vi "Lidar_obstacle.vi"(8 "error in (no error)":errorcluster, 10 "Enum Zone":T1, 11 "Tableau lidar":dbl[][](array[numeric])=[[0.0, 1.0, 2.0, 3.0, 4.0, 5.0, 6.0, 7.0, 8.0, 9.0, 10.0, 11.0, 12.0, 13.0, 14.0, 15.0, 16.0, 17.0, 18.0, 19.0, 20.0, 21.0, 22.0, 23.0, 24.0, 25.0, 26.0, 27.0, 28.0, 29.0, 30.0, 31.0, 32.0, 33.0, 34.0, 35.0], [20.0, 15.0, 30.0, 31.0, 42.0, 50.0, 51.0, 60.0, 20.0, 15.0, 30.0, 31.0, 42.0, 50.0, 51.0, 60.0, 20.0, 15.0, 30.0, 31.0, 42.0, 50.0, 51.0, 60.0, 20.0, 15.0, 30.0, 31.0, 42.0, 50.0, 51.0, 60.0, 20.0, 15.0, 30.0, 31.0], [0.0, 0.0, 0.0, 0.0, 0.0, 0.0, 0.0, 0.0, 0.0, 0.0, 0.0, 0.0, 0.0, 0.0, 0.0, 0.0, 0.0, 0.0, 0.0, 0.0, 0.0, 0.0, 0.0, 0.0, 0.0, 0.0, 0.0, 0.0, 0.0, 0.0, 0.0, 0.0, 0.0, 0.0, 0.0, 0.0]]) -> (0 "error out":errorcluster, 1 "Zone 2":dbl[][](array[numeric]), 2 "Zone 3":dbl[][](array[numeric]), 3 "Espace libre":dbl[][](array[numeric]))   [LabVIEW 2018]
uses:
  enum_zone.ctl
panel:
  out "Espace libre sans angle visé":dbl[][](array[numeric])
  out "Index ZM":i32
  out "Ecart superieur Alpha":dbl[][](array[numeric])
  out "Zone 3 bis + limite ZM":dbl[][](array[numeric])
  out "initialized array ecart":dbl[][](array[numeric])
  out "Zone 3 Bis":dbl[][](array[numeric])
  out "Detec part 3":dbl[][](array[numeric])
  out "Nbr ° à enlever début 2":i32
  out "Nbr ° à enlever fin 2":i32
  out "Début detec 3":i32
  out "Detec part 4":dbl[][](array[numeric])
  out "Moitié de Alpha":dbl
  in  "Alpha":i32=90
  in  "L2":dbl=30.0
  in  "L3":dbl=60.0
  out "Zone de detection":dbl[][](array[numeric])
  out "Nbr ° à enlever fin":dbl
  out "Début detec 2":dbl
  out "Detec part 2":dbl[][](array[numeric])
  out "Nbr ° à enlever début":dbl
  out "Detec part 1":dbl[][](array[numeric])
  out "Moitié de ZM":dbl
  in  "Angle zone morte (°)":i32=180
  out "Angles / distance / statut":dbl[][](array[numeric])
  # "Face Avant"
  # "Debug"
  # "Zone morte retirée"
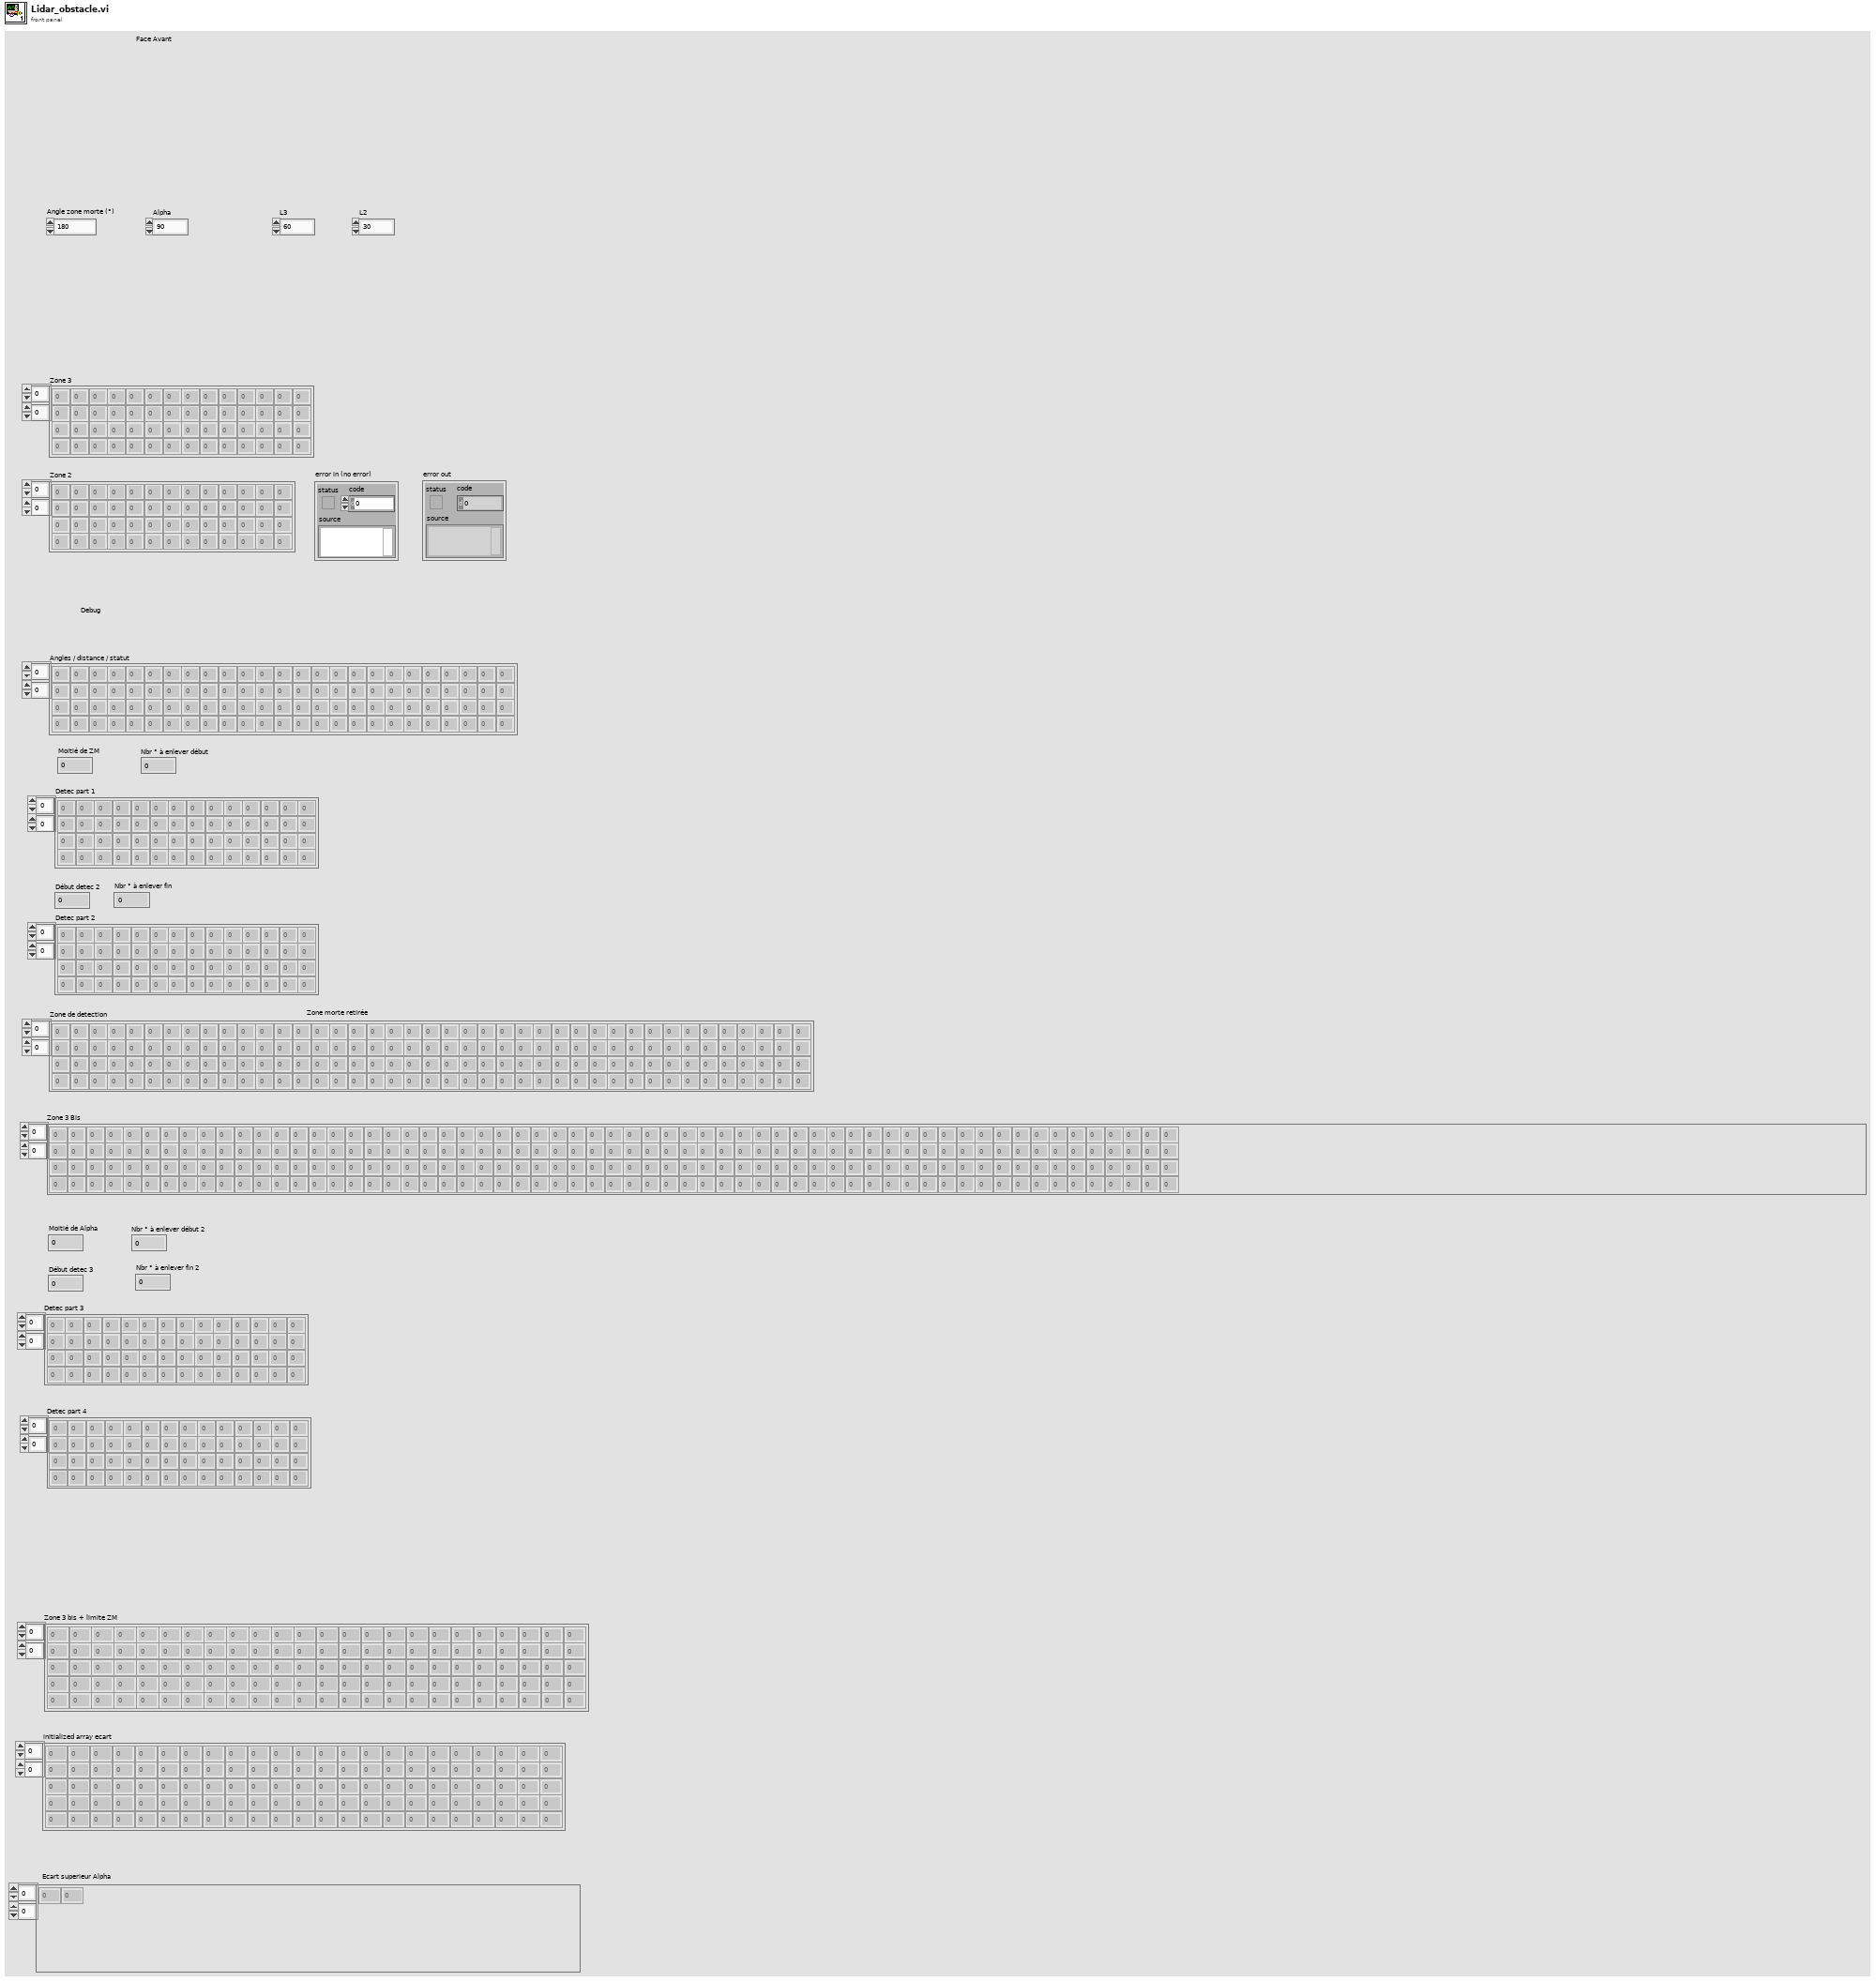
[diagram p1: front panel]
types:
  T1 = typedef "enum_zone.ctl" = enum16{"Zone_2", "Zone_3", "Espace_libre", "Aucune"}
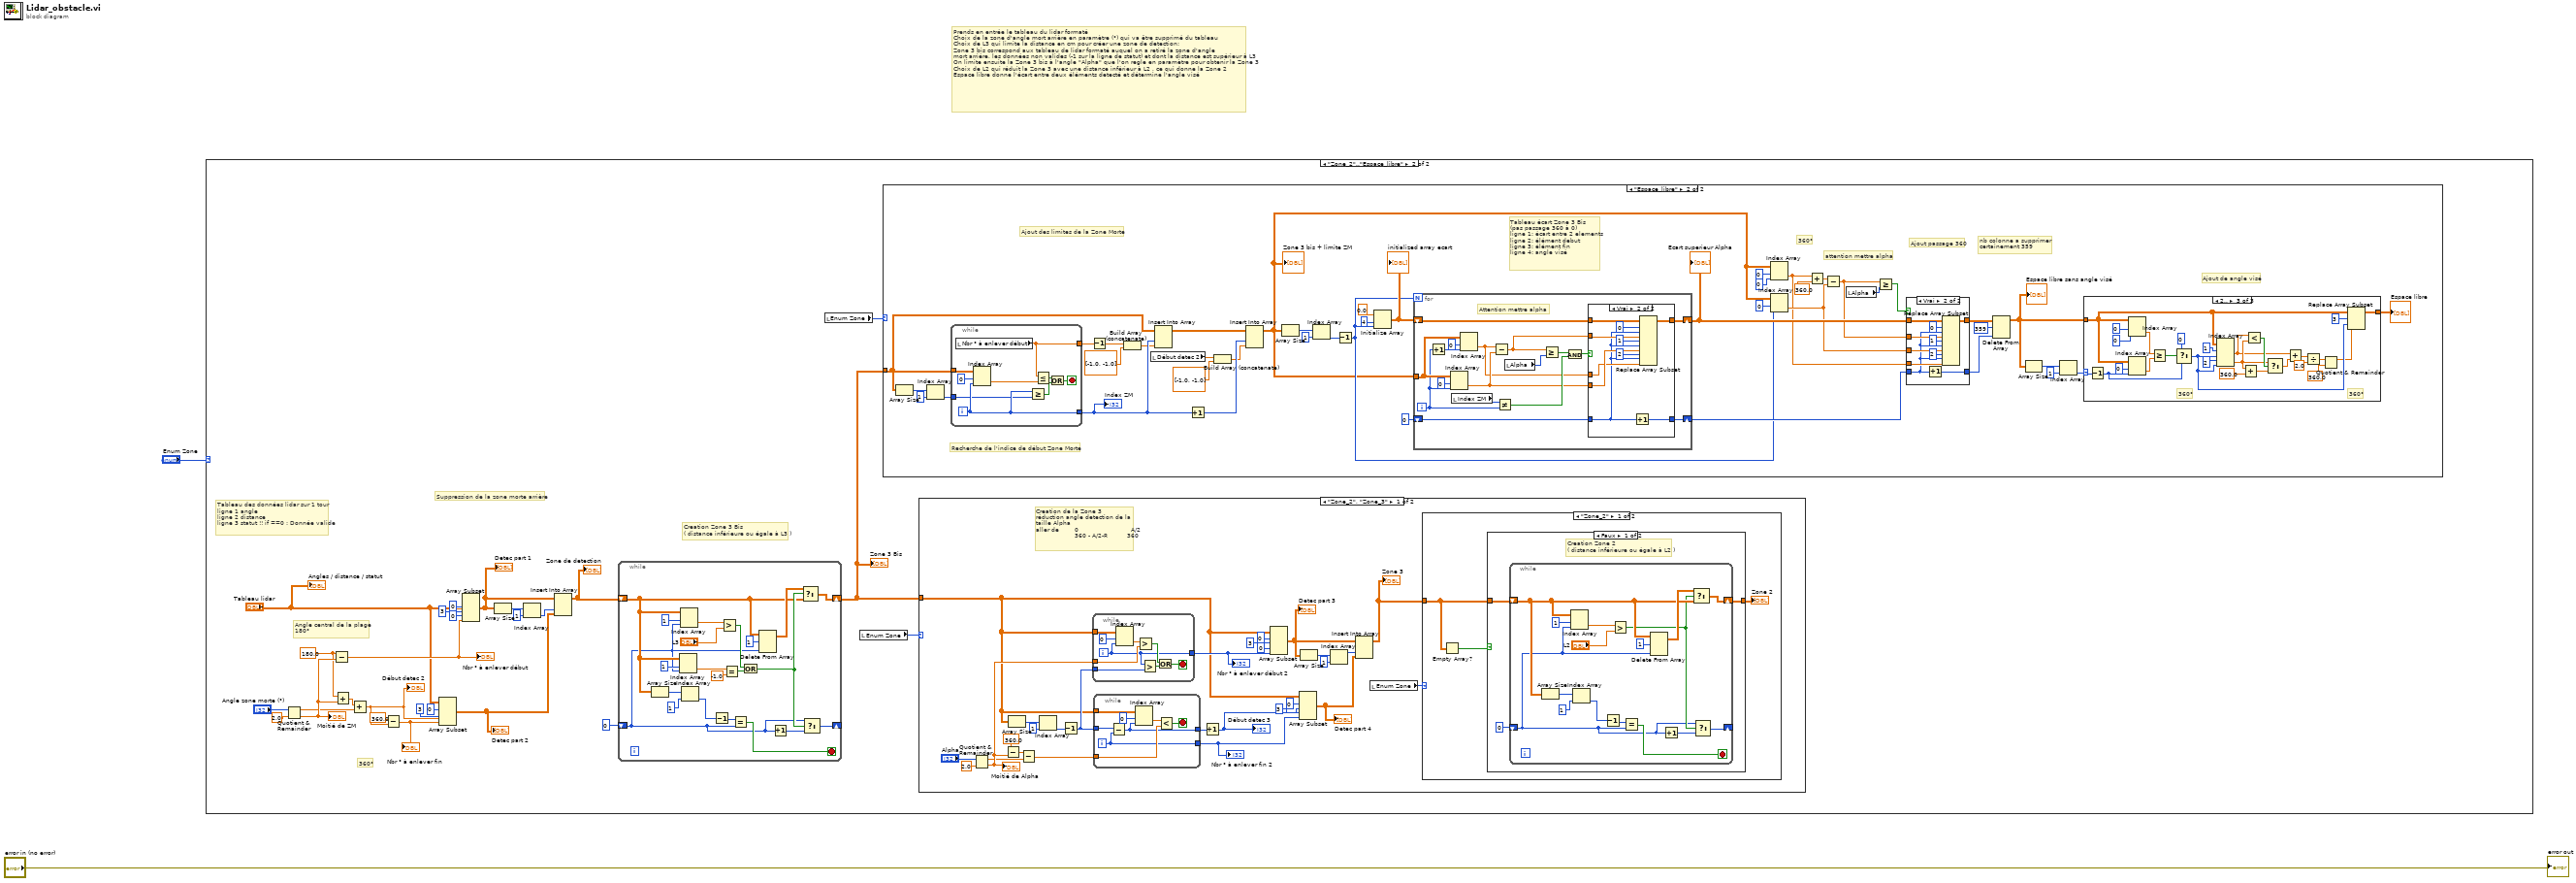
[diagram p0: block diagram]
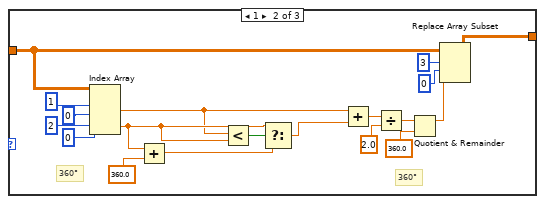
[diagram p5: hidden frame]
diagram:
  # "Prends en entrée le tableau du lidar formaté\nChoix de la zone d'angle mort arrière en paramètre (°) qui va être supprimé du tableau\nChoix de L3 qui limite la distance en cm pour créer une zone de detection:\nZone 3 bis correspond aux tableau de lidar formaté auquel on a retiré la zone d'angle\nmort arriére, les données non valides (-1 sur la ligne de statut) et dont la distance est supérieur à L3\nOn limite ensuite la Zone 3 bis à l'angle \"Alpha\" que l'on regle en paramètre pour obtenir la Zone 3\nChoix de L2 qui réduit la Zone 3 avec une distance inférieur à L2 , ce qui donne la Zone 2\nEspace libre donne l'écart entre deux éléments detecté et détermine l'angle visé"
  n1 = case shown="\"Zone_2\"..\"Espace_libre\"" "Enum Zone" {
    frame "Aucune", Default {
    }
    frame "Zone_2".."Espace_libre" {
      w8 = 180.0 ("x")
      # "360°"
      # "Creation Zone 3 Bis \n( distance inférieure ou égale à L3 )"
      # "Angle central de la plage\n180°"
      # "Suppression de la zone morte arrière"
      # "Tableau des données lidar sur 1 tour\nligne 1 angle\nligne 2 distance\nligne 3 statut !! if ==0 : Donnée valide"
      n2 = Quotient & Remainder(x="Angle zone morte (°)", y=2.0) -> (x-y*floor(x/y)=w17:dbl, floor(x/y)=w26:dbl)
      "Moitié de ZM" <- w26
      n3 = Subtract(x=w8, y=w26) -> (x-y=w7:dbl)
      "Nbr ° à enlever début" <- w7
      n4 = Add(x=w8, y=w26) -> (x+y=w18:dbl)
      n5 = Add(x=w18, y=w17) -> (x+y=w11:dbl)
      "Début detec 2" <- w11
      n6 = Subtract(x=360.0, y=w11) -> (x-y=w24:dbl)
      "Nbr ° à enlever fin" <- w24
      n7 = Array Subset(array="Tableau lidar", index (row)=0 ("index"), length (row)=3 ("length"), index (col)=w11, length (col)=w24) -> (w13:dbl[][])
      "Detec part 2" <- w13
      n8 = Array Subset(array="Tableau lidar", index (row)=0 ("index"), length (row)=3 ("length"), index (col)=0 ("index"), length (col)=w7) -> (w14:dbl[][])
      "Detec part 1" <- w14
      n9 = Array Size(array=w14) -> (size(s)=w16:i32[])
      n10 = Index Array(array=w16, index=1) -> (element=w12:i32)
      n11 = Insert Into Array(array=w14, index (col)=w12, new element=w13) -> (w9:dbl[][])  [unwired: 1 in]
      "Zone de detection" <- w9
      n12 = while {
        shift-right: [w248] -> w6
        shift-left: w9 -> [w238]
        shift-right: [w250] -> _
        shift-left: 0 -> [w237]
        stop <- w247 stop-if-true
        n13 = Array Size(array=w238) -> (size(s)=w252:i32[])
        n14 = Index Array(array=w238, index (row)=1 ("disabled index (row)"), index (col)=w237) -> (element=w236:dbl)
        n15 = Index Array(array=w238, index (row)=1 ("disabled index (row)"), index (col)=w237) -> (element=w254:dbl)
        n16 = Index Array(array=w252, index=1) -> (element=w245:i32)
        n17 = Decrement(x=w245) -> (x-1=w246:i32)
        n18 = Greater?(x=w254, y="L3") -> (0:w241:bool)
        n19 = Equal?(x=w236, y=-1.0) -> (x = y?=w242:bool)
        n20 = Equal?(x=w246, y=w237) -> (x = y?=w247:bool)
        n21 = Or(x=w241, y=w242) -> (x .or. y?=w243:bool)
        n22 = Delete From Array(array=w238, length=1, index (col)=w237) -> (array with subset deleted=w253:dbl[][])  [unwired: 1 in, 1 out]
        n23 = Increment(x=w237) -> (x+1=w249:i32)
        n24 = Select(t=w253, s=w243, f=w238) -> (s? t:f=w248:dbl[][])
        n25 = Select(t=w237, s=w243, f=w249) -> (s? t:f=w250:i32)
      }
      "Zone 3 Bis" <- w6
      n26 = local read "Enum Zone"() -> (w5:T1)
      n27 = local read "Enum Zone"() -> (w4:T1)
      n28 = case shown="\"Espace_libre\"" w5 {
        tunnel: w6 -> [_ w30]
        frame "Zone_2", "Zone_3", "Aucune", Default {
        }
        frame "Espace_libre" {
          # "Recherche de l'indice de début Zone Morte"
          # "nb colonne a supprimer\ncertainement 359"
          # "360°"
          # "Ajout des limites de la Zone Morte"
          # "Ajout de angle visé"
          # "attention mettre alpha"
          # "Ajout passage 360"
          # "Tableau écart Zone 3 Bis\n(pas passage 360 à 0)\nligne 1: écart entre 2 elements\nligne 2: élément debut\nligne 3: élément fin\nligne 4: angle visé"
          n29 = Array Size(array=w30) -> (size(s)=w32:i32[])
          n30 = Index Array(array=w32, index=1) -> (element=w29:i32)
          n31 = while {
            tunnel: w30 -> [w167]
            tunnel: [w160] -> w64
            tunnel: [w164] -> w63
            tunnel: w29 -> [w159]
            i -> [w160]
            stop <- w162 stop-if-true
            n32 = local read "Nbr ° à enlever début"() -> (w164:dbl)
            n33 = Index Array(array=w167, index (row)=0 ("disabled index (row)"), index (col)=w160) -> (element=w165:dbl)
            n34 = Greater Or Equal?(x=w160, y=w159) -> (x >= y?=w161:bool)
            n35 = Less Or Equal?(x=w164, y=w165) -> (x <= y?=w163:bool)
            n36 = Or(x=w163, y=w161) -> (x .or. y?=w162:bool)
          }
          "Index ZM" <- w64
          n37 = Decrement(x=w63) -> (x-1=w62:dbl)
          n38 = Build Array (concatenate)(w62, dbl[] [-1.0, -1.0] ("array")) -> (w61:dbl[])
          n39 = local read "Début detec 2"() -> (w57:dbl)
          n40 = Insert Into Array(array=w30, index (col)=w64, new element=w61) -> (w66:dbl[][])  [unwired: 1 in]
          n41 = Increment(x=w64) -> (x+1=w65:i32)
          n42 = Build Array (concatenate)(w57, dbl[] [-1.0, -1.0] ("array")) -> (w58:dbl[])
          n43 = Insert Into Array(array=w66, index (col)=w65, new element=w58) -> (w47:dbl[][])  [unwired: 1 in]
          "Zone 3 bis + limite ZM" <- w47
          n44 = Array Size(array=w47) -> (size(s)=w69:i32[])
          n45 = Index Array(array=w69, index=1) -> (element=w67:i32)
          n46 = Decrement(x=w67) -> (x-1=w48:i32)
          n47 = Initialize Array(0.0 ("element"), 4 ("dimension size"), w48) -> (w56:dbl[][])
          "initialized array ecart" <- w56
          n48 = for {
            N: w48 -> [_]
            tunnel: w47 -> [w145]
            shift-right: [w138] -> w53
            shift-left: w56 -> [w137]
            shift-right: [w133] -> w52
            shift-left: 0 -> [w134]
            i -> [w136]
            # "Attention mettre alpha"
            n49 = Increment(x=w136) -> (x+1=w142:i32)
            n50 = Index Array(array=w145, index (row)=0, index (col)=w136) -> (element=w132:dbl)
            n51 = local read "Index ZM"() -> (w140:i32)
            n52 = Index Array(array=w145, index (row)=0, index (col)=w142) -> (element=w131:dbl)
            n53 = Subtract(x=w131, y=w132) -> (x-y=w135:dbl)
            n54 = Not Equal?(x=w140, y=w136) -> (x != y?=w139:bool)
            n55 = local read "Alpha"() -> (w130:i32)
            n56 = Greater Or Equal?(x=w135, y=w130) -> (x >= y?=w141:bool)
            n57 = And(x=w141, y=w139) -> (x .and. y?=w146:bool)
            n58 = case shown="Vrai" w146 {
              tunnel: [w148 w156] -> w138
              tunnel: w137 -> [w148 w157]
              tunnel: w135 -> [_ w153]
              tunnel: w134 -> [w147 w149]
              tunnel: [w147 w158] -> w133
              tunnel: w132 -> [_ w151]
              tunnel: w131 -> [_ w150]
              frame False {
              }
              frame True {
                n59 = Increment(x=w149) -> (x+1=w158:i32)
                n60 = Replace Array Subset(array=w157, new element #1=w153, index (row) #1=0 ("index (row)"), index (col) #1=w149, new element #2=w151, index (row) #2=1 ("disabled index (row)"), index (col) #2=w149, new element #3=w150, index (row) #3=2 ("disabled index (row)"), index (col) #3=w149) -> (w156:dbl[][])
              }
            }
          }
          "Ecart superieur Alpha" <- w53
          n61 = Index Array(array=w47, index (row)=0, index (col)=0) -> (element=w41:dbl)
          n62 = Index Array(array=w47, index (row)=0, index (col)=w48) -> (element=w42:dbl)
          n63 = Add(x=w41, y=360.0) -> (x+y=w45:dbl)
          n64 = Subtract(x=w45, y=w42) -> (x-y=w43:dbl)
          n65 = local read "Alpha"() -> (w33:i32)
          n66 = Greater Or Equal?(x=w43, y=w33) -> (x >= y?=w44:bool)
          n67 = case shown="Vrai" w44 {
            tunnel: w53 -> [w119 w129]
            tunnel: w52 -> [w118 w121]
            tunnel: w43 -> [_ w125]
            tunnel: w42 -> [_ w124]
            tunnel: w41 -> [_ w123]
            tunnel: [w119 w122] -> w40
            tunnel: [w118 w120] -> w39
            frame False {
            }
            frame True {
              n68 = Increment(x=w121) -> (x+1=w120:i32)
              n69 = Replace Array Subset(array=w129, new element #1=w125, index (row) #1=0 ("disabled index (row)"), index (col) #1=w121, new element #2=w124, index (row) #2=1 ("disabled index (row)"), index (col) #2=w121, new element #3=w123, index (row) #3=2 ("disabled index (row)"), index (col) #3=w121) -> (w122:dbl[][])
            }
          }
          n70 = Delete From Array(array=w40, length=359, index (col)=w39) -> (array with subset deleted=w35:dbl[][])  [unwired: 1 in, 1 out]
          "Espace libre sans angle visé" <- w35
          n71 = Array Size(array=w35) -> (size(s)=w38:i32[])
          n72 = Index Array(array=w38, index=1) -> (element=w36:i32)
          n73 = case shown="2.." w36 {
            selector: w36 -> [_ _ w117]
            tunnel: w35 -> [w72 w82 w103]
            tunnel: [w72 w83 w99] -> w34
            frame 0, Default {
            }
            frame 1 {
              # "360°"
              # "360°"
              n74 = Index Array(array=w82, index (row) #1=1 ("index (row)"), index (col) #1=0 ("disabled index (col)"), index (row) #2=2 ("index (row)"), index (col) #2=0 ("disabled index (col)")) -> (element #1=w73:dbl, element #2=w74:dbl)
              n75 = Add(x=w74, y=360.0) -> (x+y=w76:dbl)
              n76 = Less?(x=w73, y=w74) -> (x < y?=w75:bool)
              n77 = Select(t=w74, s=w75, f=w76) -> (s? t:f=w77:dbl)
              n78 = Add(x=w73, y=w77) -> (x+y=w89:dbl)
              n79 = Divide(x=w89, y=2.0) -> (x/y=w87:dbl)
              n80 = Quotient & Remainder(x=w87, y=360.0) -> (x-y*floor(x/y)=w84:dbl)  [unwired: 1 out]
              n81 = Replace Array Subset(array=w82, new element=w84, index (row)=3, index (col)=0) -> (w83:dbl[][])
            }
            frame 2.. {
              # "360°"
              # "360°"
              n82 = Decrement(x=w117) -> (x-1=w110:i32)
              n83 = Index Array(array=w103, index (row)=0, index (col)=0 ("disabled index (col)")) -> (element=w113:dbl)
              n84 = Index Array(array=w103, index (row)=0 ("disabled index (row)"), index (col)=w110) -> (element=w112:dbl)
              n85 = Greater Or Equal?(x=w113, y=w112) -> (x >= y?=w96:bool)
              n86 = Select(t=0, s=w96, f=w110) -> (s? t:f=w101:i32)
              n87 = Index Array(array=w103, index (row) #1=1 ("index (row)"), index (col) #1=w101, index (row) #2=2 ("index (row)"), index (col) #2=w101) -> (element #1=w92:dbl, element #2=w93:dbl)
              n88 = Add(x=w93, y=360.0) -> (x+y=w97:dbl)
              n89 = Less?(x=w92, y=w93) -> (x < y?=w94:bool)
              n90 = Select(t=w93, s=w94, f=w97) -> (s? t:f=w95:dbl)
              n91 = Add(x=w92, y=w95) -> (x+y=w107:dbl)
              n92 = Divide(x=w107, y=2.0) -> (x/y=w105:dbl)
              n93 = Quotient & Remainder(x=w105, y=360.0) -> (x-y*floor(x/y)=w100:dbl)  [unwired: 1 out]
              n94 = Replace Array Subset(array=w103, new element=w100, index (row)=3, index (col)=w101) -> (w99:dbl[][])
            }
          }
          "Espace libre" <- w34
        }
      }
      n95 = case shown="\"Zone_2\", \"Zone_3\"" w4 {
        tunnel: w6 -> [w169 _]
        frame "Zone_2", "Zone_3" {
          # "Creation de la Zone 3\nréduction angle detection de la taille Alpha\naller de        0                           A/2\n                    360 - A/2-R          360"
          n96 = Quotient & Remainder(x="Alpha", y=2.0) -> (x-y*floor(x/y)=w180:dbl, floor(x/y)=w194:dbl)
          "Moitié de Alpha" <- w194
          n97 = Subtract(x=360.0, y=w194) -> (x-y=w179:dbl)
          n98 = Array Size(array=w169) -> (size(s)=w181:i32[])
          n99 = Subtract(x=w179, y=w180) -> (x-y=w183:dbl)
          n100 = Index Array(array=w181, index=1) -> (element=w182:i32)
          n101 = Decrement(x=w182) -> (x-1=w187:i32)
          n102 = while {
            tunnel: w169 -> [w212]
            tunnel: w194 -> [w210]
            tunnel: [w205] -> w190
            tunnel: w187 -> [w204]
            i -> [w205]
            stop <- w207 stop-if-true
            n103 = Index Array(array=w212, index (row)=0, index (col)=w205) -> (element=w209:dbl)
            n104 = Greater?(x=w209, y=w210) -> (0:w208:bool)
            n105 = Greater?(x=w205, y=w204) -> (0:w206:bool)
            n106 = Or(x=w208, y=w206) -> (x .or. y?=w207:bool)
          }
          "Nbr ° à enlever début 2" <- w190
          n107 = while {
            tunnel: w169 -> [w202]
            tunnel: w187 -> [w201]
            tunnel: w183 -> [w199]
            tunnel: [w198] -> w184
            tunnel: [w197] -> w191
            i -> [w197]
            stop <- w196 stop-if-true
            n108 = Subtract(x=w201, y=w197) -> (x-y=w198:i32)
            n109 = Index Array(array=w202, index (row)=0, index (col)=w198) -> (element=w200:dbl)
            n110 = Less?(x=w200, y=w199) -> (x < y?=w196:bool)
          }
          "Nbr ° à enlever fin 2" <- w191
          n111 = Increment(x=w184) -> (x+1=w192:i32)
          "Début detec 3" <- w192
          n112 = Array Subset(array=w169, index (row)=0 ("index"), length (row)=3 ("length"), index (col)=0 ("index"), length (col)=w190) -> (w188:dbl[][])
          "Detec part 3" <- w188
          n113 = Array Subset(array=w169, index (row)=0 ("index"), length (row)=3 ("length"), index (col)=w192, length (col)=w191) -> (w189:dbl[][])
          "Detec part 4" <- w189
          n114 = Array Size(array=w188) -> (size(s)=w185:i32[])
          n115 = Index Array(array=w185, index=1) -> (element=w186:i32)
          n116 = Insert Into Array(array=w188, index (col)=w186, new element=w189) -> (w168:dbl[][])  [unwired: 1 in]
          "Zone 3" <- w168
          n117 = local read "Enum Zone"() -> (w195:T1)
          n118 = case shown="\"Zone_2\"" w195 {
            tunnel: w168 -> [w213 _]
            frame "Zone_2" {
              n119 = Empty Array?(array=w213) -> (empty?=w214:bool)
              n120 = case shown="Faux" w214 {
                tunnel: w213 -> [w217 w235]
                tunnel: [w216 w235] -> w215
                frame False {
                  # "Creation Zone 2\n( distance inférieure ou égale à L2 )"
                  n121 = while {
                    shift-right: [w224] -> w216
                    shift-left: w217 -> [w228]
                    shift-right: [w226] -> _
                    shift-left: 0 -> [w222]
                    stop <- w223 stop-if-true
                    n122 = Array Size(array=w228) -> (size(s)=w230:i32[])
                    n123 = Index Array(array=w228, index (row)=1 ("disabled index (row)"), index (col)=w222) -> (element=w232:dbl)
                    n124 = Index Array(array=w230, index=1) -> (element=w220:i32)
                    n125 = Decrement(x=w220) -> (x-1=w221:i32)
                    n126 = Greater?(x=w232, y="L2") -> (0:w227:bool)
                    n127 = Equal?(x=w221, y=w222) -> (x = y?=w223:bool)
                    n128 = Delete From Array(array=w228, length=1, index (col)=w222) -> (array with subset deleted=w231:dbl[][])  [unwired: 1 in, 1 out]
                    n129 = Increment(x=w222) -> (x+1=w225:i32)
                    n130 = Select(t=w231, s=w227, f=w228) -> (s? t:f=w224:dbl[][])
                    n131 = Select(t=w222, s=w227, f=w225) -> (s? t:f=w226:i32)
                  }
                }
                frame True {
                }
              }
              "Zone 2" <- w215
            }
            frame "Zone_3".."Aucune", Default {
            }
          }
        }
        frame "Espace_libre", "Aucune", Default {
        }
      }
      "Angles / distance / statut" <- "Tableau lidar"
    }
  }
  "error out" <- "error in (no error)"
